vi "Scalar Template.vi"   [LabVIEW 2012]
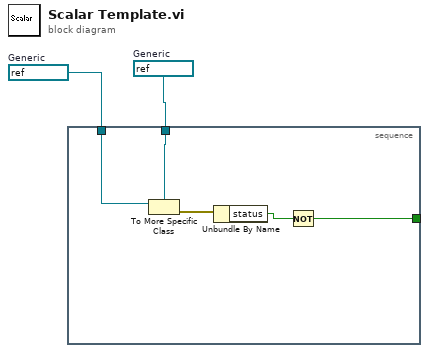
[diagram p0: block diagram]
diagram:
  w2 = refnum<vi> refnum  # Generic
  w1 = refnum<vi> refnum  # Generic
  n1 = stacked-sequence {
    tunnel: [w3] -> _
    tunnel: w2 -> [w5]
    tunnel: w1 -> [w4]
    frame #0 {
      n2 = To More Specific Class(target class=w5, reference=w4) -> (error out=w7:errorcluster)  [unwired: 1 in, 1 out]
      n3 = Unbundle By Name(w7) -> ("status"=w6:bool)
      n4 = Not(x=w6) -> (.not. x?=w3:bool)
    }
  }
